vi "Zolix Connect.vi"() -> ()   [LabVIEW 2026, in "UI-Zolix.lvlib"]
uses:
  <vilib>/ptbypt/NI_PtbyPt.lvlib
panel:
  in  "Calib(+)":dbl[](array[numeric])
  out "error out":errorcluster
  out "Data Out":dbl[](array[numeric]) format="%.2f"
  in  "VISA资源名称":refnum<visa-resource-name>
  in  "错误输入（无错误）":errorcluster
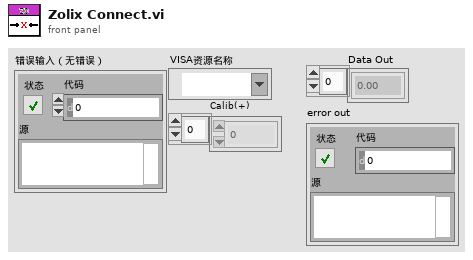
[diagram p1: front panel]
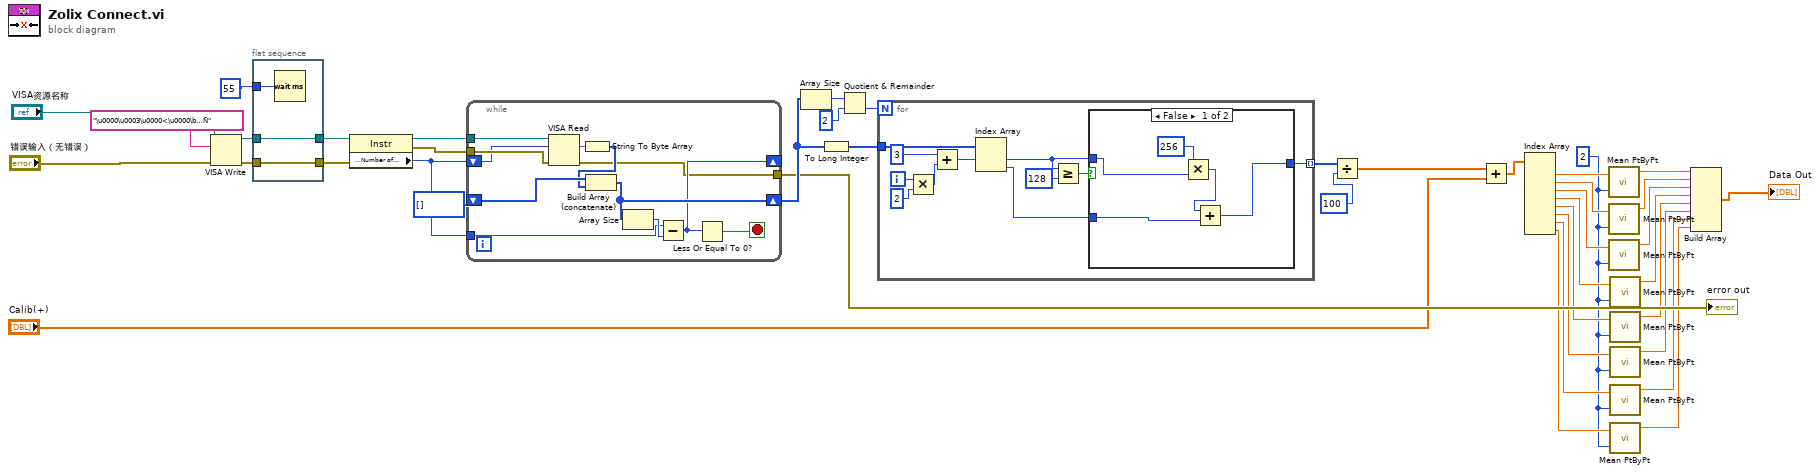
[diagram p0: block diagram]
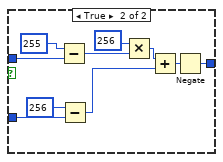
[diagram p2: hidden frame]
diagram:
  w3 = 2 ("sample length")
  n1 = VISA Write(VISA resource name="VISA资源名称", write buffer="\u0000\u0003\u0000<\u0000\b…Ñ" ("Command"), error in (no error)="错误输入（无错误）") -> (VISA resource name out=w39:refnum<visa-resource-name>, error out=w41:errorcluster)  [unwired: 1 out]
  n2 = flat-sequence {
    tunnel: w41 -> [w43]
    tunnel: [w43] -> w40
    tunnel: w39 -> [w42]
    tunnel: [w42] -> w38
    tunnel: u32 55 ("读取前延时(ms)") -> [w44]
    frame #0 {
      n3 = Wait (ms)(milliseconds to wait=w44) -> ()  [unwired: 1 out]
    }
  }
  n4 = property class="Instr"(reference=w38, error in=w40) -> (reference out=w29:refnum<visa-resource-name>, error out=w28:errorcluster, "Serial Settings:Number of Bytes at Serial Port"=w27:u32)
  n5 = while {
    tunnel: w29 -> [w54]
    tunnel: w28 -> [w53]
    shift-right: [w56] -> w34
    shift-left: u8[] [] ("unsigned byte array") -> [w55]
    tunnel: w27 -> [w48]
    shift-right: [w46] -> _
    shift-left: w27 -> [w52]
    tunnel: [w45] -> w22
    stop <- w47 stop-if-true
    n6 = VISA Read(VISA resource name=w54, byte count=w52, error in (no error)=w53) -> (read buffer=w51:string, error out=w45:errorcluster)  [unwired: 2 out]
    n7 = String To Byte Array(string=w51) -> (unsigned byte array=w50:u8[])
    n8 = Build Array (concatenate)(w55, w50) -> (w56:u8[])
    n9 = Array Size(array=w56) -> (size(s)=w49:i32)
    n10 = Subtract(x=w48, y=w49) -> (x-y=w46:u32)
    n11 = Less Or Equal To 0?(x=w46) -> (x <= 0?=w47:bool)
  }
  "error out" <- w22
  n12 = Array Size(array=w34) -> (size(s)=w32:i32)
  n13 = To Long Integer(number=w34) -> (32bit integer=w35:i32[])
  n14 = Quotient & Remainder(x=w32, y=2) -> (floor(x/y)=w31:i32)  [unwired: 1 out]
  n15 = for {
    N: w31 -> [_]
    tunnel: w35 -> [w67]
    tunnel: [w57] -> w23 mode=indexing
    i -> [w64]
    n16 = Multiply(x=w64, y=2) -> (x*y=w62:i32)
    n17 = Add(x=3 ("索引"), y=w62) -> (x+y=w65:i32)
    n18 = Index Array(array=w67, index #1=w65) -> (element #1=w59:i32, element #2=w58:i32)  [unwired: 1 in]
    n19 = Greater Or Equal?(x=w59, y=128) -> (x >= y?=w61:bool)
    n20 = case shown="False" w61 {
      tunnel: w59 -> [w71 w80]
      tunnel: w58 -> [w69 w78]
      tunnel: [w68 w73] -> w57
      frame False {
        n21 = Multiply(x=256, y=w71) -> (x*y=w72:i32)
        n22 = Add(x=w72, y=w69) -> (x+y=w68:i32)
      }
      frame True {
        n23 = Subtract(x=255, y=w80) -> (x-y=w77:i32)
        n24 = Subtract(x=256, y=w78) -> (x-y=w75:i32)
        n25 = Multiply(x=256, y=w77) -> (x*y=w76:i32)
        n26 = Add(x=w76, y=w75) -> (x+y=w74:i32)
        n27 = Negate(x=w74) -> (-x=w73:i32)
      }
    }
  }
  n28 = Divide(x=w23, y=100) -> (x/y=w21:dbl[])
  n29 = Add(x=w21, y="Calib(+)") -> (x+y=w2:dbl[])
  n30 = Index Array(array=w2) -> (element #1=w19:dbl, element #2=w18:dbl, element #3=w17:dbl, element #4=w16:dbl, element #5=w15:dbl, element #6=w14:dbl, element #7=w13:dbl, element #8=w12:dbl)  [unwired: 8 in]
  n31 = call <vilib>:"Mean PtByPt.vi"("x"=w19, "sample length"=w3) -> ("mean"=w11:dbl)  [unwired: 2 in, 1 out]
  n32 = call <vilib>:"Mean PtByPt.vi"("x"=w18, "sample length"=w3) -> ("mean"=w10:dbl)  [unwired: 2 in, 1 out]
  n33 = call <vilib>:"Mean PtByPt.vi"("x"=w17, "sample length"=w3) -> ("mean"=w9:dbl)  [unwired: 2 in, 1 out]
  n34 = call <vilib>:"Mean PtByPt.vi"("x"=w16, "sample length"=w3) -> ("mean"=w8:dbl)  [unwired: 2 in, 1 out]
  n35 = call <vilib>:"Mean PtByPt.vi"("x"=w15, "sample length"=w3) -> ("mean"=w7:dbl)  [unwired: 2 in, 1 out]
  n36 = call <vilib>:"Mean PtByPt.vi"("x"=w14, "sample length"=w3) -> ("mean"=w6:dbl)  [unwired: 2 in, 1 out]
  n37 = call <vilib>:"Mean PtByPt.vi"("x"=w13, "sample length"=w3) -> ("mean"=w5:dbl)  [unwired: 2 in, 1 out]
  n38 = call <vilib>:"Mean PtByPt.vi"("x"=w12, "sample length"=w3) -> ("mean"=w4:dbl)  [unwired: 2 in, 1 out]
  n39 = Build Array(w11, w10, w9, w8, w7, w6, w5, w4) -> (→"Data Out":dbl[])
